vi "Update Scrollbars.vi"(8 "error in (no error)":errorcluster, 11 "2DArrayManager in":refnum<class "2DArrayManager.lvclass">) -> (0 "error out":errorcluster, 3 "2DArrayManager out":refnum<class "2DArrayManager.lvclass">)   [LabVIEW 2020, in "OOPanel.lvlib" / "2DArrayManager.lvclass"]
uses:
  2DArrayManager.lvclass
  2DArrayManager.lvclass/2DArrayManager.ctl
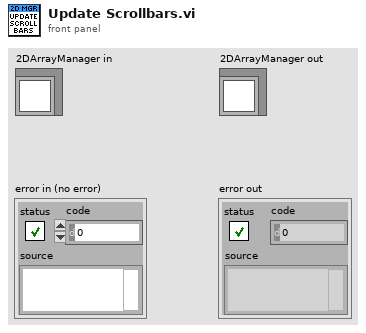
[diagram p1: front panel]
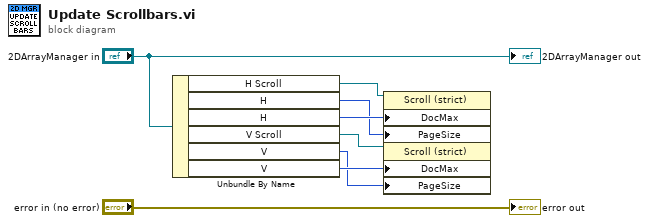
[diagram p0: block diagram]
diagram:
  n1 = Unbundle By Name("2DArrayManager in") -> ("H Scroll"=w4:refnum<vi>, "H"=w1:i32, "H"=w2:i32, "V Scroll"=w5:refnum<vi>, "V"=w3:i32, "V"=w6:i32)
  n2 = property class="Scroll (strict)"(reference=w4, "DocMax"=w2, "PageSize"=w1) -> ()  [unwired: 1 in, 2 out]
  n3 = property class="Scroll (strict)"(reference=w5, "DocMax"=w6, "PageSize"=w3) -> ()  [unwired: 1 in, 2 out]
  "error out" <- "error in (no error)"
  "2DArrayManager out" <- "2DArrayManager in"
